vi "D_R_Temp.vi"(8 "error in (no error)":errorcluster, 11 "bID":u8) -> (0 "error out":errorcluster, 1 "CBTemp":dbl, 2 "HeadTemp":dbl, 3 "bID":u8, 4 "TorF":i32)   [LabVIEW 2017]
uses:
  LabVIEW2018/hpkSLMdaLV.dll
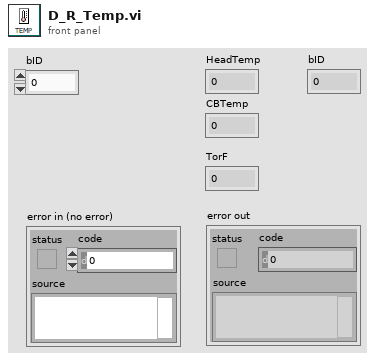
[diagram p1: front panel]
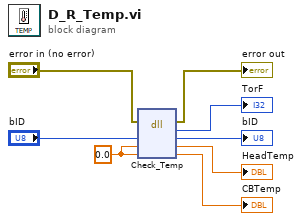
[diagram p0: block diagram]
diagram:
  w5 = 0.0 ("headTemp")
  n1 = dll-call lib="C:/Users/hs5921/Desktop/LabVIEW2018/hpkSLMdaLV.dll" fn="Check_Temp"(error in="error in (no error)", "bID"="bID", "headTemp"=w5, "CBTemp"=w5) -> (error out=→"error out":errorcluster, "返り値タイプ"=→"TorF":i32, "bID"=→"bID":u8, "headTemp"=→"HeadTemp":dbl, "CBTemp"=→"CBTemp":dbl)  [unwired: 2 in, 1 out]
